vi "GDM-9052 Read Frequery(Voltage).vi"() -> ()   [LabVIEW 2021, in "GDM-9052.lvlib"]
uses:
  GDM-9052.lvlib
panel:
  in  "Manual Range":dbl format="%#.9e"
  in  "Configure RS232 Baud Rate":u32(ring)=115200 items=["9600"=9600, "19200"=19200, "38400"=38400, "57600"=57600, "115200"=115200]
  out "error out":errorcluster
  out "Measure Value":string
  in  "Stop":bool
  out "Boolean":bool
  in  "Detector Rate":u16(ring) items=["SLOW", "MID", "FAST"]
  in  "Enable Auto Range":bool=TRUE
  out "ID Return String":string
  in  "VISA resource name":refnum<visa-resource-name>
  # "GDM-9052 Read Frequery(Voltage)"
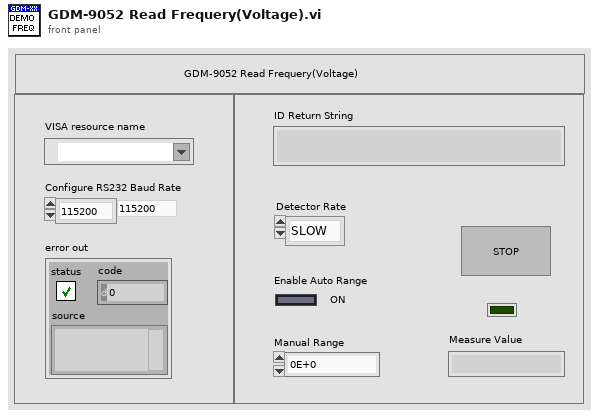
[diagram p1: front panel]
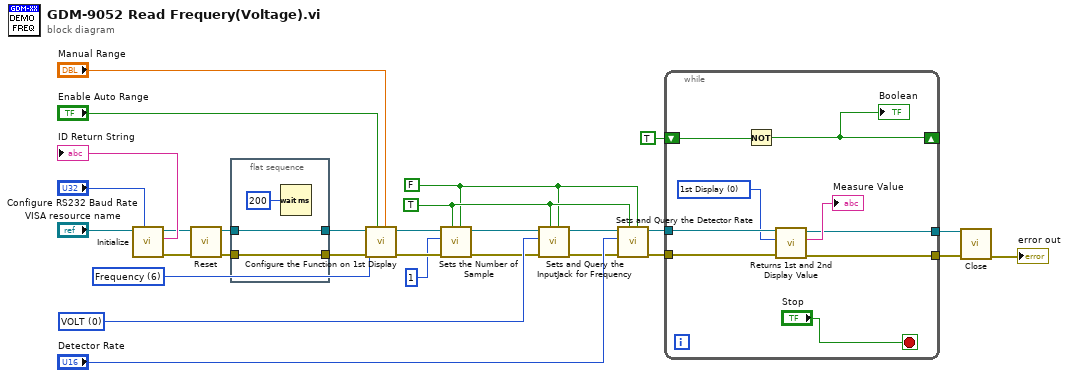
[diagram p0: block diagram]
diagram:
  w2 = u8 6 items=["DC Voltage", "AC Voltage", "DC Current", "AC Current", "2-Wire Resistance", "4-Wire Resistance", "Frequency", "Period", "Continuity", "Diode", "Temperature", "Capacitance"] ("Function")
  w11 = u8 0 items=["VOLT", "500mA", "10A"] ("Input Jack")
  w5 = FALSE ("Enable to Query")
  w6 = TRUE ("Enable to Sets")
  n1 = call "Initialize.vi"("Configure RS232 Baud Rate"="Configure RS232 Baud Rate", "VISA resource name"="VISA resource name") -> ("error out"=w19:errorcluster, "ID Return String"=→"ID Return String":string, "VISA resource name out"=w20:refnum<visa-resource-name>)  [unwired: 6 in, 1 out]
  n2 = call "Reset.vi"("error in (no error)"=w19, "VISA resource name"=w20) -> ("error out"=w15:errorcluster, "VISA resource name out"=w17:refnum<visa-resource-name>)  [unwired: 8 in]
  n3 = flat-sequence {
    tunnel: w17 -> [w32]
    tunnel: [w32] -> w16
    tunnel: w15 -> [w31]
    tunnel: [w31] -> w14
    frame #0 {
      n4 = Wait (ms)(milliseconds to wait=u32 200) -> ()  [unwired: 1 out]
    }
  }
  n5 = call "Configure the Function on 1st Display .vi"("Manual Range"="Manual Range", "Enable Auto Range"="Enable Auto Range", "error in"=w14, "Function"=w2, "VISA resource name"=w16) -> ("error out"=w7:errorcluster, "VISA resource name out"=w10:refnum<visa-resource-name>)  [unwired: 5 in]
  n6 = call "Sets the Number of Sample.vi"("Enable to Query"=w5, "Enable to Sets"=w6, "error in"=w7, "Number of Sample"=u16 1, "VISA resource name"=w10) -> ("error out"=w8:errorcluster, "VISA resource name out"=w9:refnum<visa-resource-name>)  [unwired: 4 in, 1 out]
  n7 = call "Sets and Query the InputJack for Frequency.vi"("Enable to Query"=w5, "Enable to Sets"=w6, "error in"=w8, "Input Jack"=w11, "VISA resource name"=w9) -> ("error out"=w12:errorcluster, "VISA resource name out"=w13:refnum<visa-resource-name>)  [unwired: 4 in, 1 out]
  n8 = call "Sets and Query the Detector Rate.vi"("Enable to Query"=w5, "Enable to Sets"=w6, "error in"=w12, "Detector Rate"="Detector Rate", "VISA resource name"=w13) -> ("error out"=w24:errorcluster, "VISA resource name out"=w25:refnum<visa-resource-name>)  [unwired: 4 in, 1 out]
  n9 = while {
    tunnel: w25 -> [w41]
    tunnel: w24 -> [w40]
    tunnel: [w36] -> w23
    tunnel: [w35] -> w22
    shift-right: [w33] -> _
    shift-left: TRUE -> [w34]
    stop <- "Stop" stop-if-true
    w39 = u16 0 items=["1st Display", "2nd Display", "1st & 2nd Display"] ("Sets to Display")
    n10 = Not(x=w34) -> (.not. x?=w33:bool)
    "Boolean" <- w33
    n11 = call "Returns 1st and 2nd Display Value.vi"("error in"=w40, "Sets to Display"=w39, "VISA resource name"=w41) -> ("error out"=w35:errorcluster, "Return the Value"=→"Measure Value":string, "VISA resource name out"=w36:refnum<visa-resource-name>)  [unwired: 6 in]
  }
  n12 = call "Close.vi"("error in (no error)"=w22, "VISA resource name"=w23) -> ("error out"=→"error out":errorcluster)  [unwired: 9 in]
